vi "Call Function.vi"(6 "Input String":string, 8 "error in":errorcluster, 9 "Function":string, 10 "Python Script":path, 11 "Python Caller in":refnum<class "Python Caller.lvclass">) -> (0 "error out":errorcluster, 2 "Return String":string, 3 "Python Caller out":refnum<class "Python Caller.lvclass">)   [LabVIEW 2026, in "Python Caller.lvclass"]
doc: "This VI calls the specified function from a python script. This VI can only call functions with a string input and output parameter. The function uses the tool global virtual environment."
uses:
  Python Caller.lvclass
  Python Caller.lvclass/Python Caller.ctl
  Interfaces/ILogger/ILogger Messages/Log Msg/Log Msg.lvclass/Log Msg.ctl
  <vilib>/ActorFramework/Message Enqueuer/Message Enqueuer.lvclass/Message Enqueuer.ctl
  <vilib>/ActorFramework/Message Enqueuer/Enqueue.vi
  Interfaces/ILogger/ILogger Messages/Log Msg/Log Msg.lvclass
  <vilib>/ActorFramework/Message Priority Queue/Priority Enqueue.vi
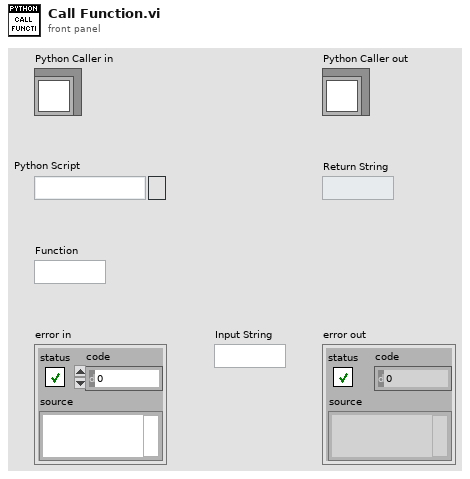
[diagram p1: front panel]
types:
  T1 = typedef "Log Entry--cluster.ctl" = cluster{"Time":timestamp, "Message":string}
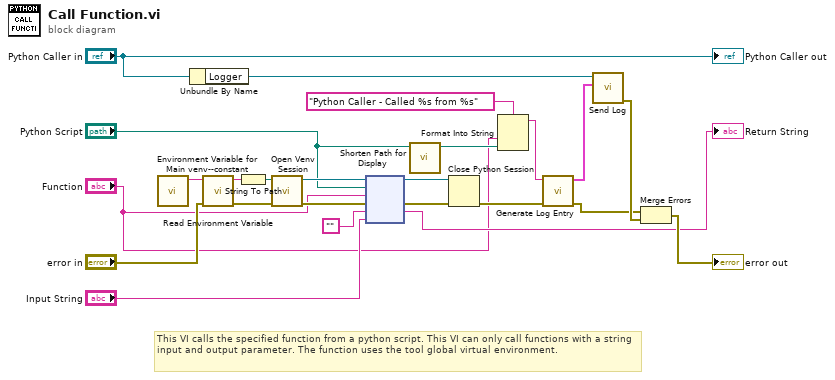
[diagram p0: block diagram]
diagram:
  # "This VI calls the specified function from a python script. This VI can only call functions with a string input and output parameter. The function uses the tool global virtual environment."
  n1 = call "Environment Variable for Main venv--constant.vi"() -> ("Environment Variable for Main venv"=w15:string)  [unwired: 11 in]
  n2 = Unbundle By Name("Python Caller in") -> ("Logger"=w7:refnum<class "Message Enqueuer.lvclass">)
  n3 = call "Read Environment Variable.vi"("error in"="error in", "Variable"=w15) -> ("error out"=w23:errorcluster, "Value"=w13:string)  [unwired: 8 in]
  n4 = String To Path(string=w13) -> (path=w14:path)
  n5 = call "Open Venv Session.vi"("error in"=w23, "Venv"=w14) -> ("error out"=w22:errorcluster, "session out"=w12:refnum<k35>)  [unwired: 8 in]
  n6 = node ("Python Node")(w12, "Python Script", "Function", w22, "" ("Empty String Constant"), "Input String") -> (w9:refnum<k35>, w21:errorcluster, →"Return String":string)  [unwired: 1 in, 2 out]
  n7 = call "Shorten Path for Display.vi"("Path"="Python Script") -> ("Shortened Path"=w2:path)  [unwired: 10 in]
  n8 = Close Python Session(session in=w9, error in=w21) -> (11:w18:errorcluster)
  n9 = Format Into String(format string="Python Caller - Called %s from %s", "Function", w2) -> (resulting string=w4:string)  [unwired: 2 in, 1 out]
  n10 = call "Generate Log Entry.vi"("error in"=w18, "Message"=w4) -> ("error out"=w17:errorcluster, "Log Entry"=w6:T1)  [unwired: 8 in]
  n11 = call "Send Log.vi"("Log Entry"=w6, "Message Enqueuer"=w7) -> ("error out"=w19:errorcluster)  [unwired: 8 in, 1 out]
  n12 = Merge Errors(w17, w19) -> (→"error out":errorcluster)
  "Python Caller out" <- "Python Caller in"
